vi "Load_ESR.vi"(8 "Tset setting( not working)":dbl=800.0, 9 "N per point":i32=7, 10 "wait time adjustment (inverted)":dbl, 11 "wait time adjustment":dbl) -> (0 "Unaveraged data":string[][](array[string]), 1 "Array":string[][](array[string]), 2 "Data":string[][](array[string]))   [LabVIEW 2024]
panel:
  in  "T set":string="5E3"
  in  "Power in dbm":string="15"
  in  "Invert pass?":bool=TRUE
  out "Passes":i32
  in  "How many passes?":i32=3
  out "Total Points":dbl
  in  "Step Size":string=".25"
  in  "Ending Frequency":string="3100"
  in  "Starting frequency":string="2650"
  # "A gate delay Typically at 1.25 us\nwidth 300 ns"
  # "15dbm is the max"
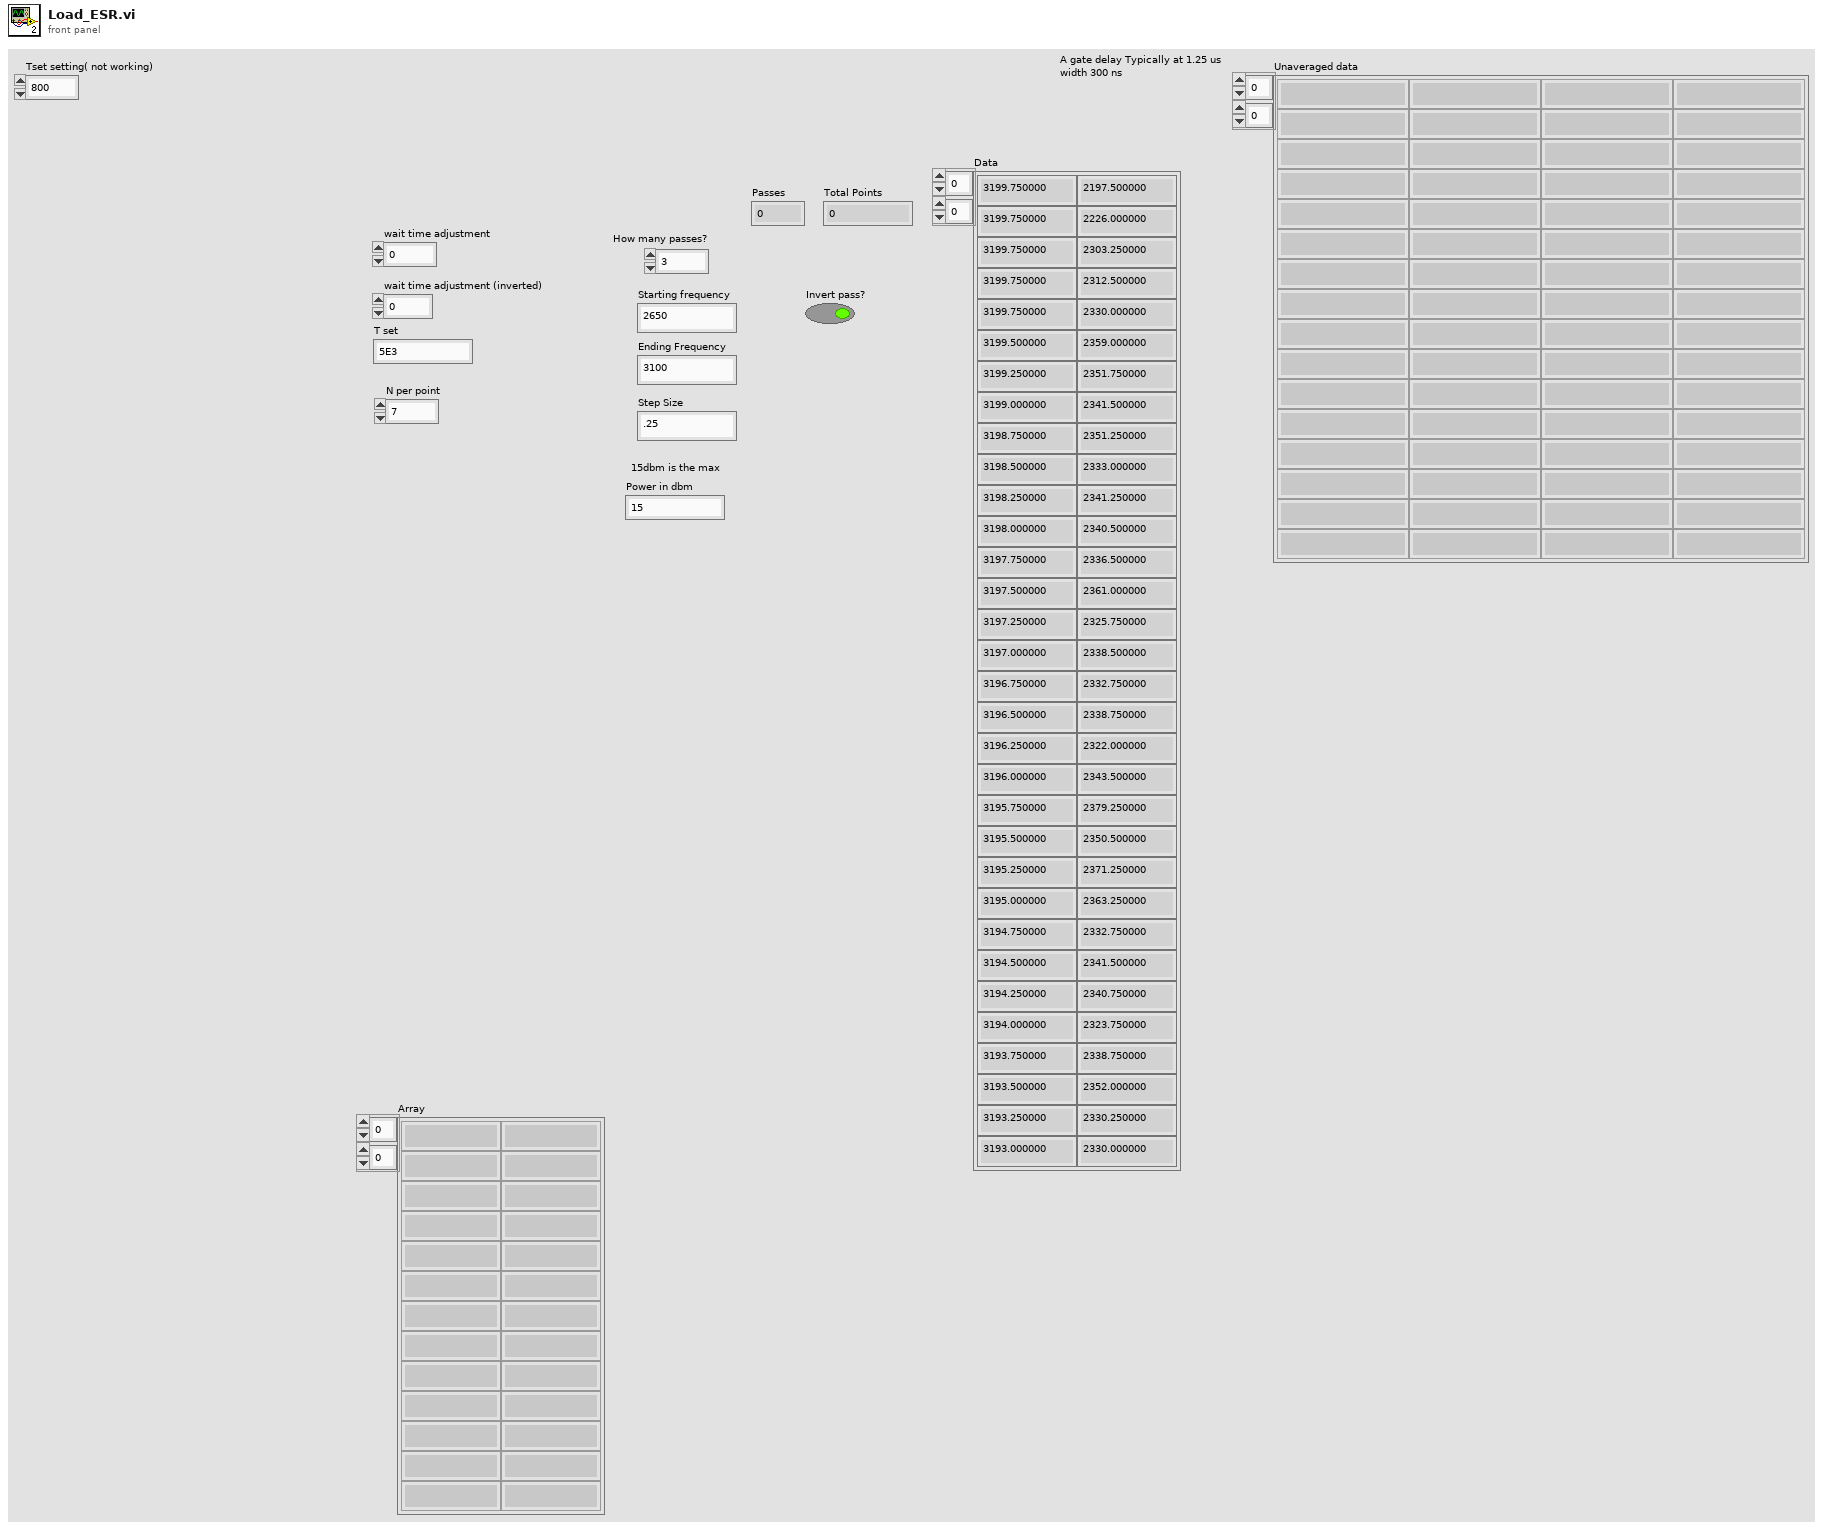
[diagram p1: front panel]
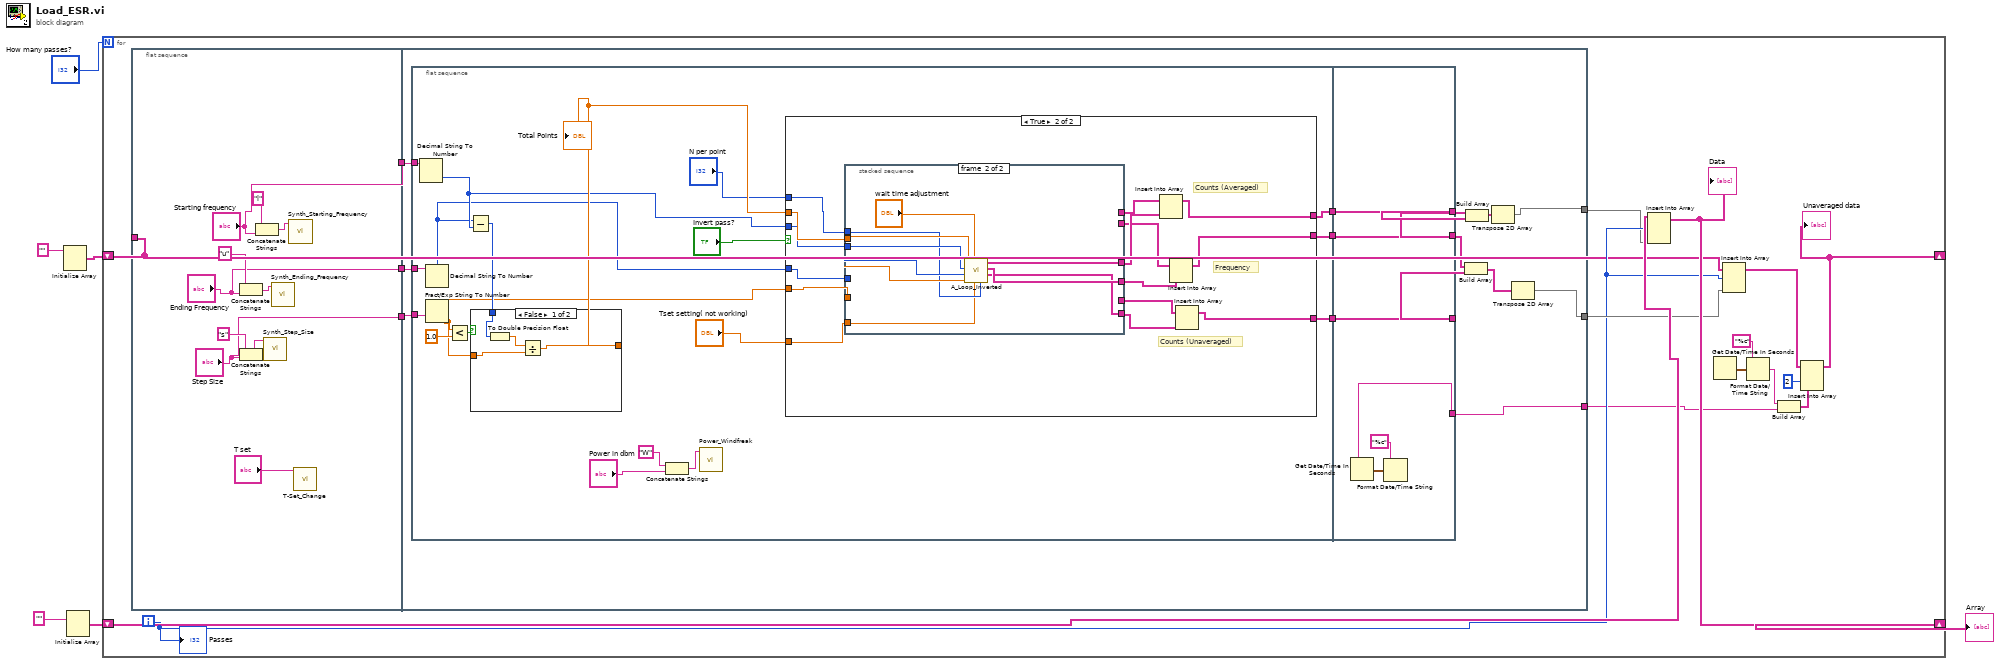
[diagram p0: block diagram]
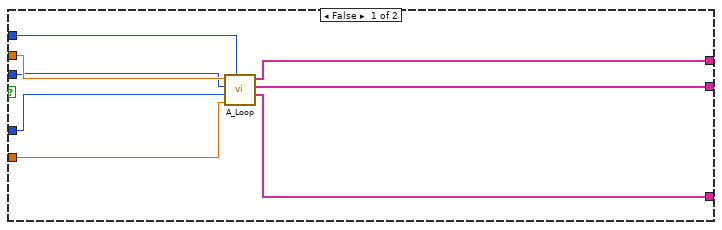
[diagram p2: hidden frame]
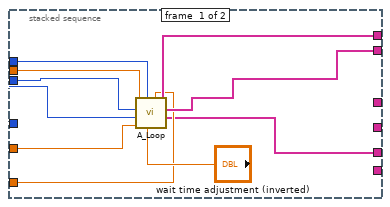
[diagram p3: hidden frame]
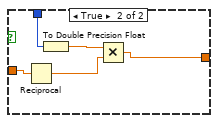
[diagram p4: hidden frame]
diagram:
  n1 = Initialize Array("") -> (w1:string[][])  [unwired: 2 in]
  n2 = Initialize Array("") -> (w4:string[][])  [unwired: 2 in]
  n3 = for {
    N: "How many passes?" -> [_]
    shift-right: [w19] -> w3
    shift-left: w4 -> [w20]
    shift-right: [w11] -> _
    shift-left: w1 -> [w10]
    i -> [w17]
    n4 = flat-sequence {
      tunnel: ["Starting frequency"] -> w23
      tunnel: ["Ending Frequency"] -> w22
      tunnel: ["Step Size"] -> w21
      tunnel: w10 -> [_]
      tunnel: w23 -> [w47]
      tunnel: w22 -> [w46]
      tunnel: w21 -> [w45]
      tunnel: [w43] -> w8
      tunnel: [w41] -> w18
      tunnel: [w34] -> w7
      frame #0 {
        n5 = Concatenate Strings("u" ("string"), "Ending Frequency") -> (w31:string)
        n6 = Concatenate Strings("s" ("string"), "Step Size") -> (w29:string)
        n7 = Concatenate Strings("l" ("string"), "Starting frequency") -> (w33:string)
        n8 = call "Synth_Step_Size.vi"("Step Size"=w29) -> ()  [unwired: 11 in]
        n9 = call "Synth_Ending_Frequency.vi"("Ending Frequency"=w31) -> ()  [unwired: 11 in]
        n10 = call "Synth_Starting_Frequency.vi"("Starting frequency"=w33) -> ()  [unwired: 11 in]
        n11 = call "T-Set_Change.vi"("T set"="T set") -> ()  [unwired: 11 in]
      }
      frame #1 {
        n12 = flat-sequence {
          tunnel: w47 -> [w66]
          tunnel: w46 -> [w65]
          tunnel: w45 -> [w63]
          tunnel: [w48] -> w37
          tunnel: [w53] -> w36
          tunnel: [w52] -> w35
          tunnel: [w122] -> w39
          tunnel: [w123] -> w40
          tunnel: [w124] -> w42
          tunnel: w37 -> [w124]
          tunnel: w36 -> [w123]
          tunnel: w35 -> [w122]
          tunnel: [w119] -> w34
          frame #0 {
            n13 = Decimal String To Number(string=w66) -> (number=w58:i32)  [unwired: 2 in, 1 out]
            n14 = Decimal String To Number(string=w65) -> (number=w57:i32)  [unwired: 2 in, 1 out]
            n15 = Fract/Exp String To Number(string=w63) -> (number=w56:dbl)  [unwired: 3 in, 1 out]
            n16 = Less?(x=w56, y=1.0) -> (x < y?=w64:bool)
            n17 = Subtract(x=w57, y=w58) -> (x-y=w61:i32)
            n18 = case shown="False" w64 {
              tunnel: w56 -> [w111 w118]
              tunnel: w61 -> [w113 w116]
              tunnel: [w110 w114] -> w59
              frame False {
                n19 = To Double Precision Float(number=w113) -> (double precision float=w112:dbl)
                n20 = Divide(x=w112, y=w111) -> (x/y=w110:dbl)
              }
              frame True {
                n21 = Reciprocal(x=w118) -> (1/x=w115:dbl)
                n22 = To Double Precision Float(number=w116) -> (double precision float=w117:dbl)
                n23 = Multiply(x=w117, y=w115) -> (x*y=w114:dbl)
              }
            }
            "Total Points" <- w59
            n24 = Concatenate Strings("W" ("string"), "Power in dbm") -> (w50:string)
            n25 = call "Power_Windfreak.vi"("Power in dbm"=w50) -> ()  [unwired: 11 in]
            n26 = case shown="True" "Invert pass?" {
              tunnel: w59 -> [w74 w89]
              tunnel: w58 -> [w73 w88]
              tunnel: w57 -> [w72 w87]
              tunnel: w56 -> [w71 w86]
              tunnel: [w70 w75] -> w48
              tunnel: [w69 w76] -> w53
              tunnel: "N per point" -> [w68 w83]
              tunnel: "Tset setting( not working)" -> [_ w82]
              tunnel: [w67 w77] -> w52
              frame False {
                n27 = call "A_Loop.vi"("N per point"=w68, "Numeric 4"=w71, "Numeric 3"=w72, "Numeric 2"=w73, "Numeric"=w74) -> ("Unaveraged"=w67:string[], "Frequency"=w69:string[], "Averaged"=w70:string[])  [unwired: 2 in, 2 out]
              }
              frame True {
                # "Counts (Unaveraged)"
                # "Counts (Averaged)"
                # "Frequency"
                n28 = stacked-sequence {
                  tunnel: w89 -> [w97 w104]
                  tunnel: w88 -> [w96 w105]
                  tunnel: w87 -> [w95 w107]
                  tunnel: w86 -> [w94 w106]
                  tunnel: [_ w109] -> w81
                  tunnel: [_ w108] -> w84
                  tunnel: [w99 _] -> w85
                  tunnel: [w98 _] -> w79
                  tunnel: w83 -> [w92 w102]
                  tunnel: w82 -> [w91 w101]
                  tunnel: [_ w100] -> w78
                  tunnel: [w90 _] -> w80
                  frame #0 {
                    n29 = call "A_Loop.vi"("Tset setting"=w91, "x"="wait time adjustment (inverted)", "N per point"=w92, "Numeric 4"=w94, "Numeric 3"=w95, "Numeric 2"=w96, "Numeric"=w97) -> ("Unaveraged"=w90:string[], "Frequency"=w98:string[], "Averaged"=w99:string[])  [unwired: 2 out]
                  }
                  frame #1 {
                    n30 = call "A_Loop_Inverted.vi"("N per point"=w102, "Tset setting"=w101, "x"="wait time adjustment", "Numeric 4"=w106, "Numeric 3"=w107, "Numeric 2"=w105, "Numeric"=w104) -> ("Array 3"=w100:string[], "output array 2"=w108:string[], "output array"=w109:string[])  [unwired: 2 in]
                  }
                }
                n31 = Insert Into Array(array=w85, new element=w81) -> (w75:string[])  [unwired: 1 in]
                n32 = Insert Into Array "Insert Into Array"(array=w79, new element=w84) -> (w76:string[])  [unwired: 1 in]
                n33 = Insert Into Array "Insert Into Array"(array=w80, new element=w78) -> (w77:string[])  [unwired: 1 in]
              }
            }
          }
          frame #1 {
            n34 = Get Date/Time In Seconds() -> (seconds since 1Jan1904=w120:timestamp)
            n35 = Format Date/Time String(time format string (%c)="%c", seconds (now)=w120) -> (date/time string=w119:string)  [unwired: 1 in]
          }
        }
        n36 = Build Array(w40, w39) -> (w38:string[][])
        n37 = Build Array(w40, w42) -> (w44:string[][])
        n38 = Transpose 2D Array(2D array=w44) -> (transposed array=w43:string[][])
        n39 = Transpose 2D Array(2D array=w38) -> (transposed array=w41:string[][])
      }
    }
    n40 = Insert Into Array(array=w20, index (row)=w17, new element=w8) -> (w19:string[][])  [unwired: 1 in]
    "Data" <- w19
    n41 = Get Date/Time In Seconds() -> (seconds since 1Jan1904=w16:timestamp)
    n42 = Insert Into Array(array=w10, index (row)=w17, new element=w18) -> (w9:string[][])  [unwired: 1 in]
    n43 = Format Date/Time String(time format string (%c)="%c", seconds (now)=w16) -> (date/time string=w15:string)  [unwired: 1 in]
    n44 = Build Array(w15, w7) -> (w14:string[])
    n45 = Insert Into Array "Insert Into Array"(array=w9, index (col)=2 ("disabled index (col)"), new element=w14) -> (w11:string[][])  [unwired: 1 in]
    "Unaveraged data" <- w11
    "Passes" <- w17
  }
  "Array" <- w3
